vi "LEDMenu.vi"(0 "ip":string) -> ()   [LabVIEW 2024]
panel:
  in  "Direction":bool
  in  "Brightness":dbl(slide) step=1.0 scale=0.0..255.0
  in  "Speed":dbl(slide) step=1.0 scale=5.0..40.0
  in  "Length":dbl(slide) step=1.0 scale=5.0..40.0
  in  "Color":u32(colorbox)
  in  "Cancel Button":bool
  in  "OK Button":bool
  # "LED Setting Menu"
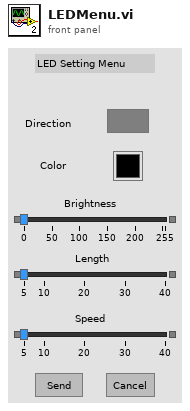
[diagram p1: front panel]
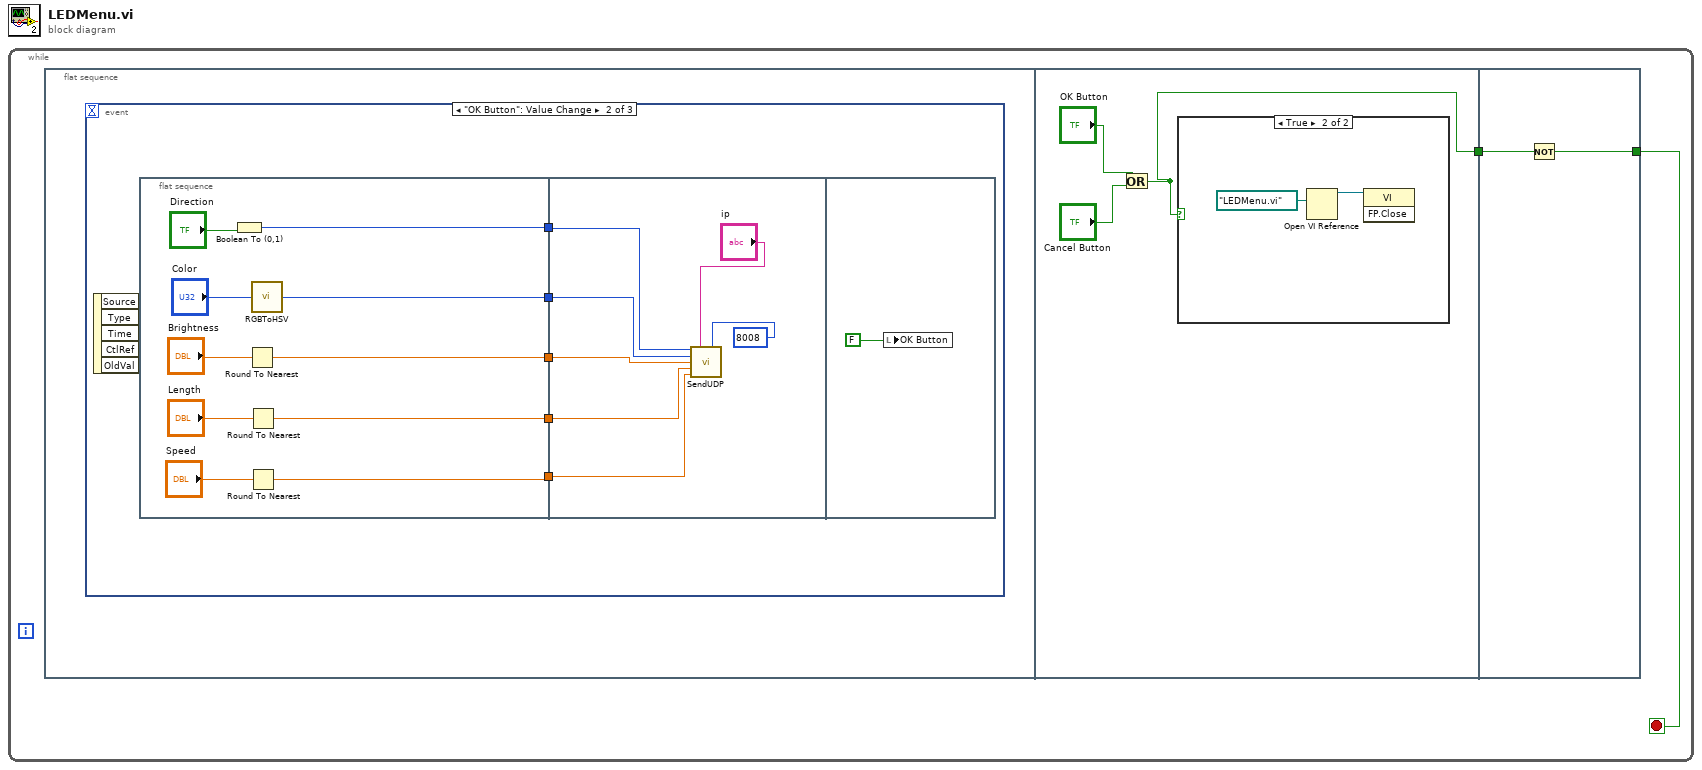
[diagram p0: block diagram]
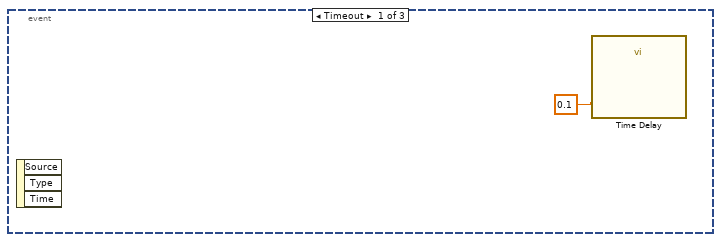
[diagram p2: hidden frame]
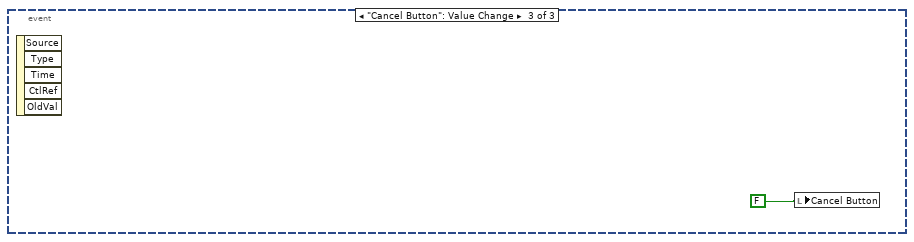
[diagram p3: hidden frame]
diagram:
  n1 = while {
    stop <- w2 stop-if-true
    n2 = flat-sequence {
      tunnel: [w28] -> w1
      tunnel: [w34] -> w2
      tunnel: w1 -> [w33]
      frame #0 {
        n3 = event shown="[1] \"OK Button\": Value Change" {
          selector: _ -> [_ _ _]
          dyn-events: _ -> [_ _ _]
          timeout: _ -> [_ _ _]
          event Timeout {
            n4 = event-data() -> ()  [unwired: 1 in, 3 out]
            n5 = call "Time Delay"("Delay Time (s)"=0.1) -> ()  [unwired: 10 in, 1 out]
          }
          event "OK Button": Value Change {
            n6 = event-data() -> ()  [unwired: 1 in, 5 out]
            n7 = flat-sequence {
              tunnel: [w17] -> w8
              tunnel: [w15] -> w7
              tunnel: [w13] -> w6
              tunnel: [w11] -> w5
              tunnel: [w9] -> w4
              tunnel: w8 -> [w23]
              tunnel: w7 -> [w22]
              tunnel: w6 -> [w21]
              tunnel: w5 -> [w20]
              tunnel: w4 -> [w19]
              frame #0 {
                n8 = Boolean To (0,1)(Boolean="Direction") -> (0, 1=w17:i16)
                n9 = Round To Nearest(number="Brightness") -> (nearest integer value=w13:dbl)
                n10 = Round To Nearest(number="Length") -> (nearest integer value=w11:dbl)
                n11 = Round To Nearest(number="Speed") -> (nearest integer value=w9:dbl)
                n12 = call "RGBToHSV.vi"("RBG U32"="Color") -> ("HSV"=w15:u16)
              }
              frame #1 {
                n13 = call "SendUDP.vi"("Arg3"=w23, "IP"="ip", "Port"=8008, "Arg4"=w22, "Arg5"=w21, "Arg6"=w20, "Arg7"=w19) -> ()  [unwired: 9 in]
              }
              frame #2 {
                n14 = local write "OK Button"(FALSE ("OK Button")) -> ()
              }
            }
          }
          event "Cancel Button": Value Change {
            n15 = event-data() -> ()  [unwired: 1 in, 5 out]
            n16 = local write "Cancel Button"(FALSE ("Cancel Button")) -> ()
          }
        }
      }
      frame #1 {
        n17 = Or(x="OK Button", y="Cancel Button") -> (x .or. y?=w28:bool)
        n18 = case shown="True" w28 {
          frame False {
          }
          frame True {
            n19 = Open VI Reference(vi path=path "LEDMenu.vi") -> (vi reference=w31:refnum<vi>)  [unwired: 5 in, 1 out]
            n20 = invoke class="VI" method="FP.Close"(reference=w31) -> ()  [unwired: 2 in, 3 out]
          }
        }
      }
      frame #2 {
        n21 = Not(x=w33) -> (.not. x?=w34:bool)
      }
    }
  }
